vi "get mcs registers.vi"(11 "MCS CSV":string[][](array[string])) -> (0 "coils":T1(array[cluster]), 1 "Array 2":i32[][](array[numeric]), 2 "Array 3":i32[][](array[numeric]), 3 "Array 4":i32[][](array[numeric]), 4 "Array":T2[][](array[typedef]))   [LabVIEW 2025]
uses:
  mcs/Tachometer_MAIN Folder/CTRLS/New/MCS Tag.ctl
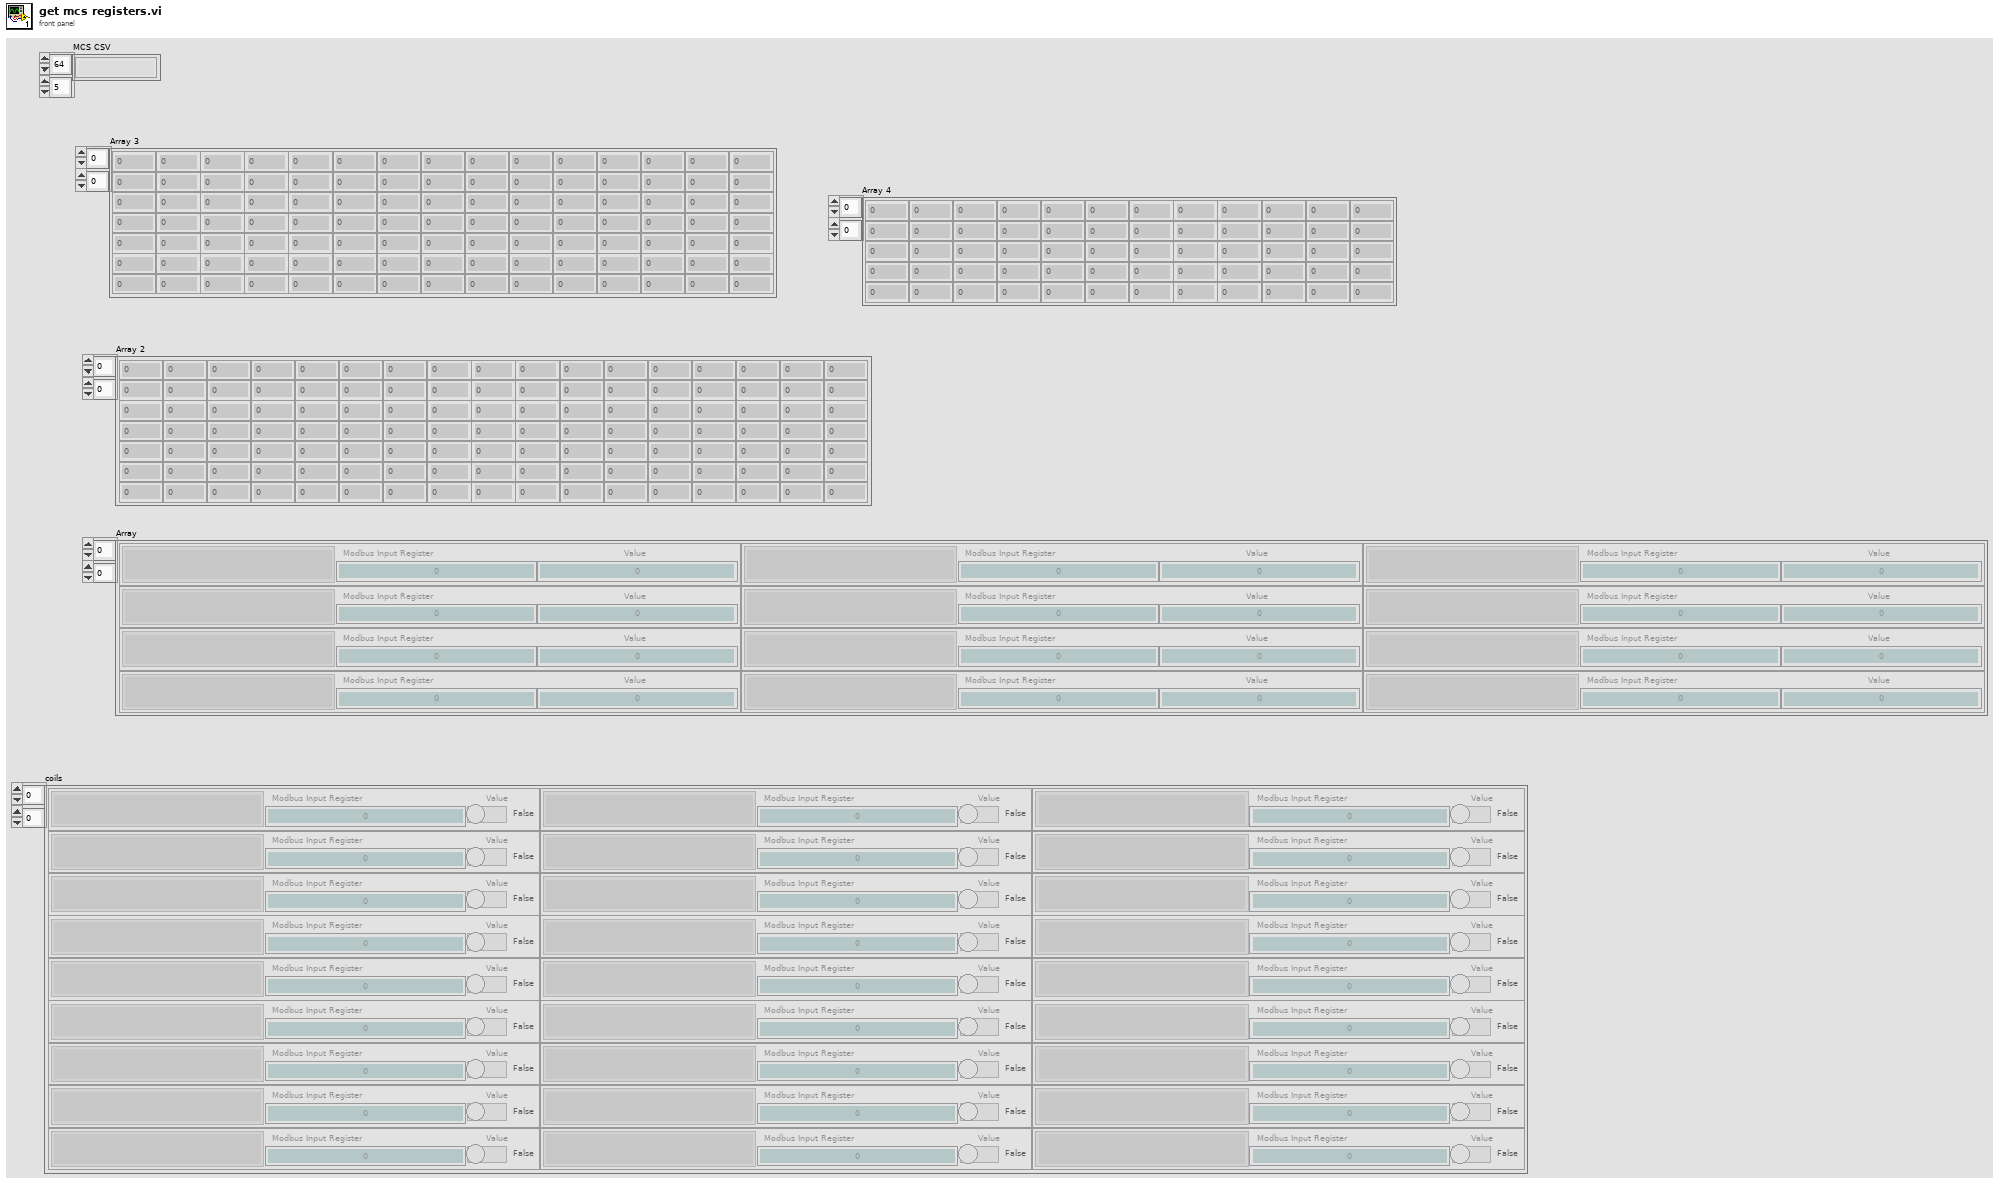
[diagram p1: front panel]
types:
  T1 = cluster{"Tag Name":string, "Modbus Input Register":sgl, "Value":bool}[][]
  T2 = typedef "MCS Tag.ctl" = cluster{"Tag Name":string, "Modbus Input Register":sgl, "Value":sgl}
  T3 = cluster{"Tag Name":string, "Modbus Input Register":sgl, bool}
  T4 = cluster{"Tag Name":string, "Modbus Input Register":sgl, bool}[]
  T5 = cluster{"Tag Name":string, "Modbus Input Register":sgl, bool}[][]
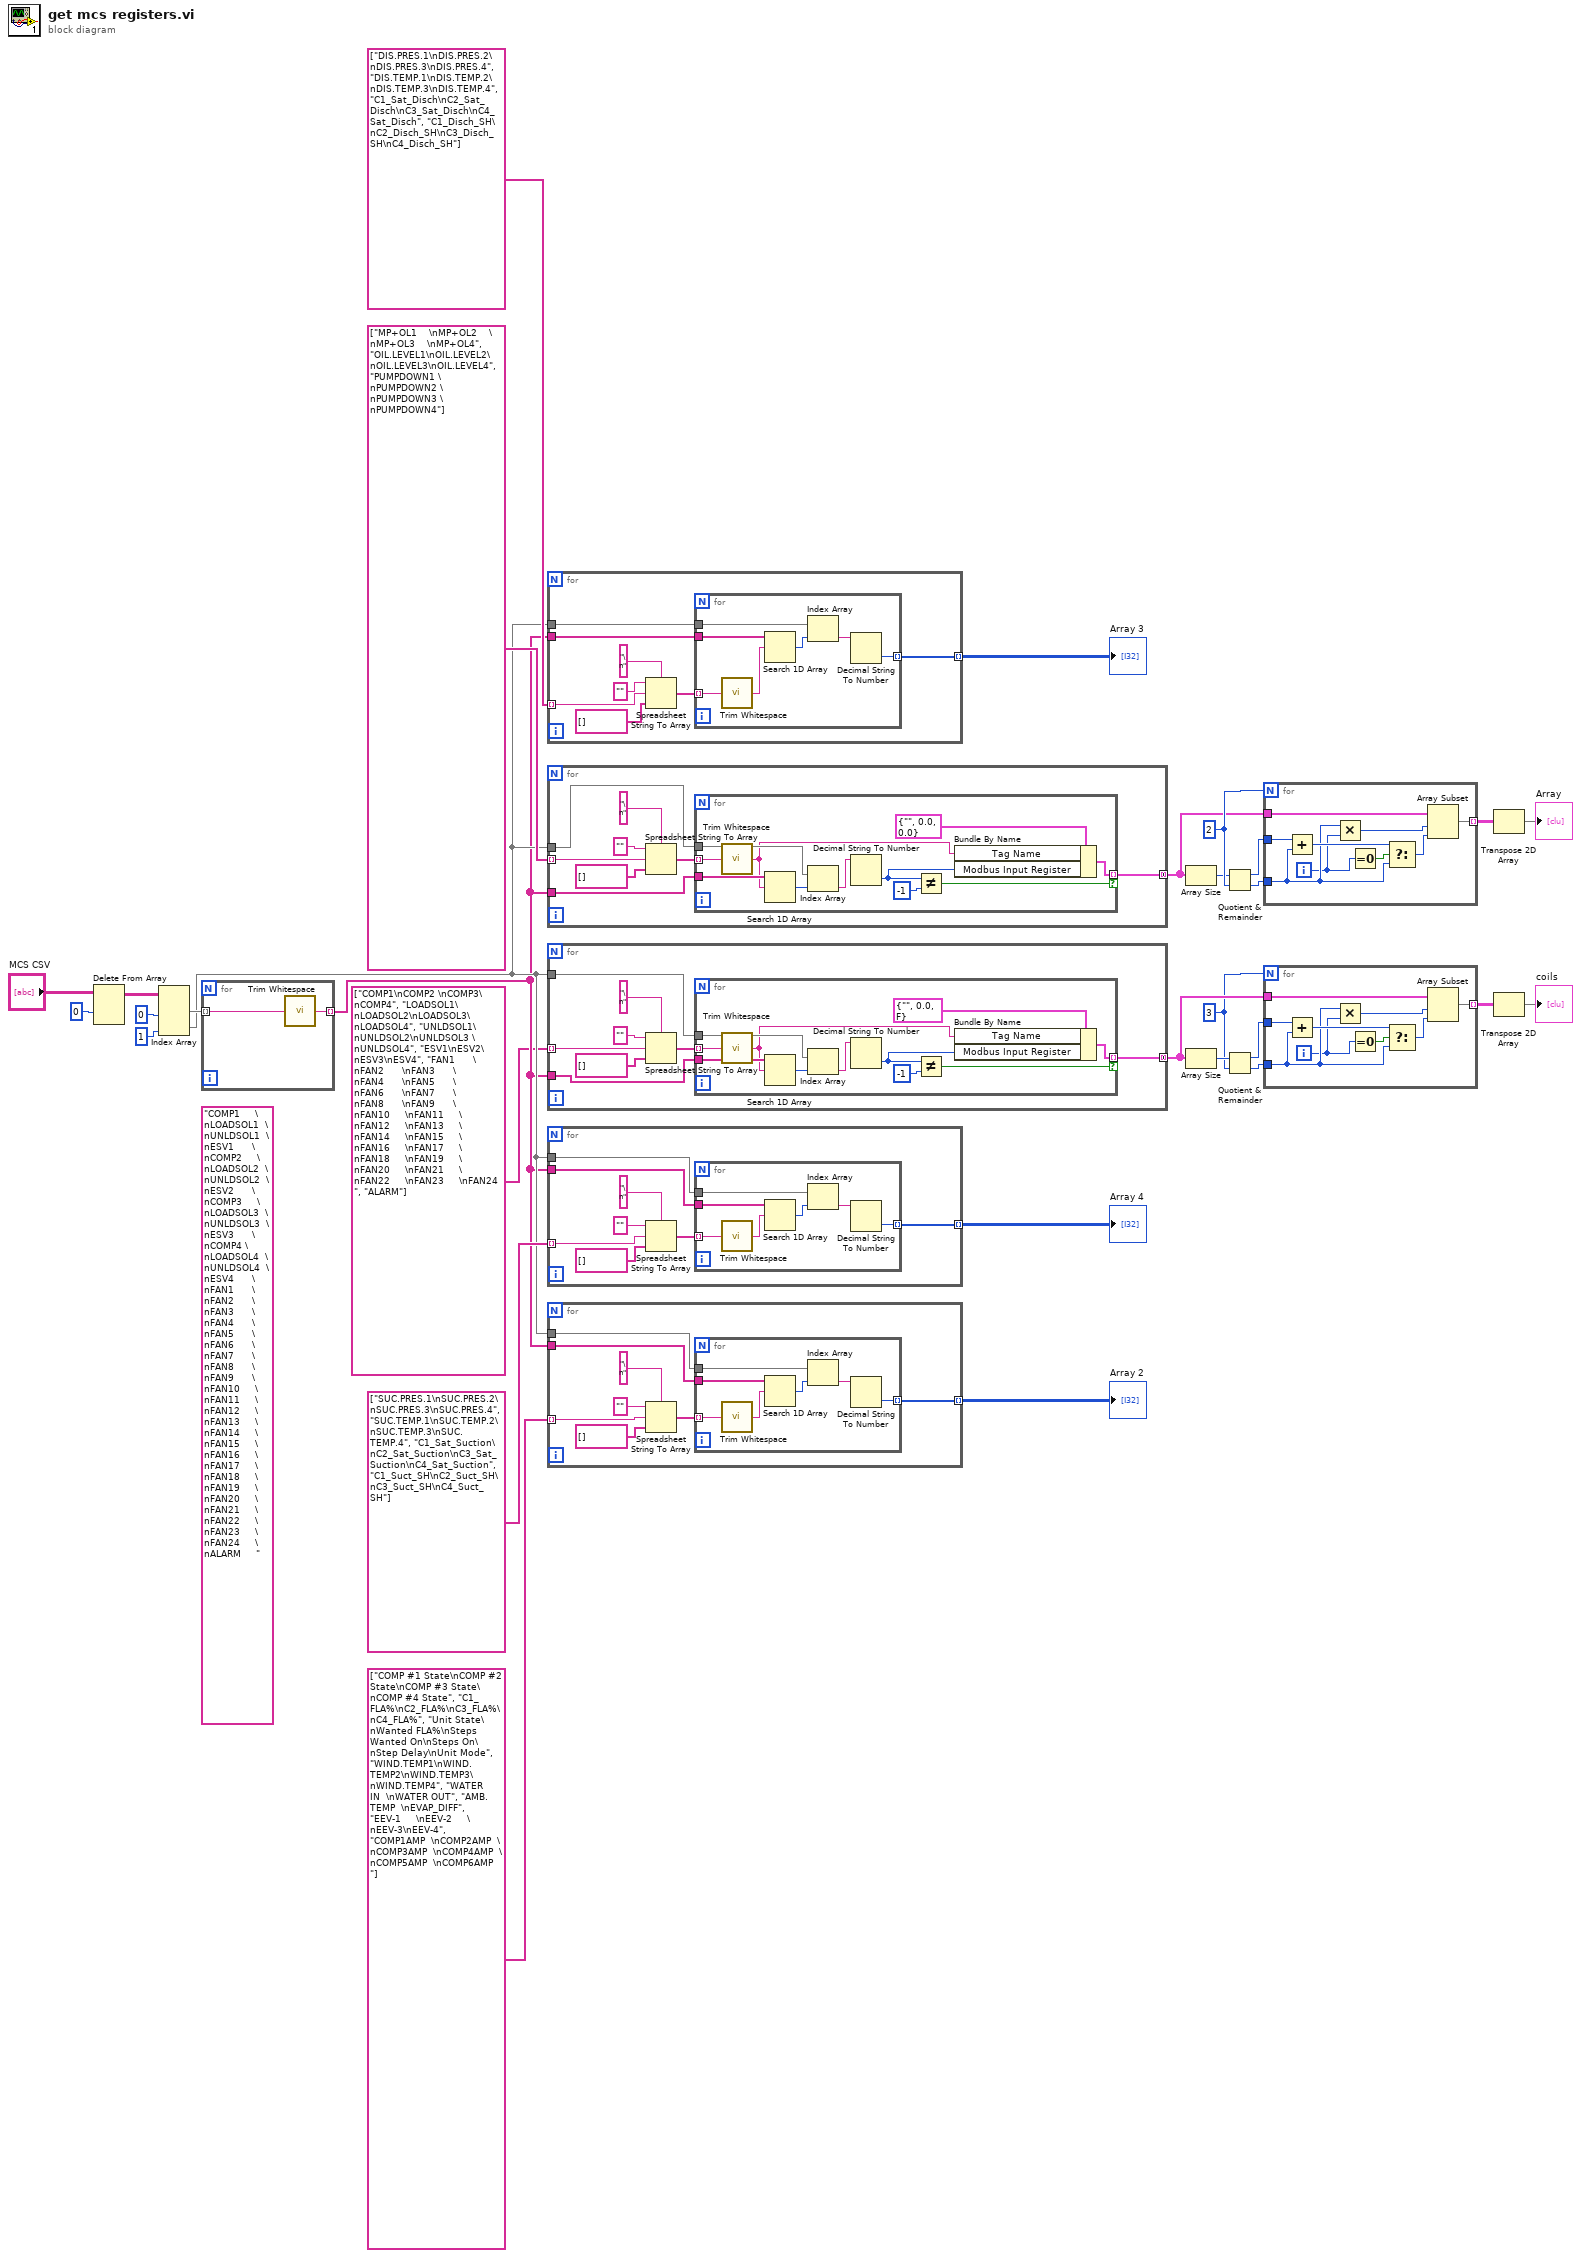
[diagram p0: block diagram]
diagram:
  w5 = 2
  w10 = 3
  (unwired) "COMP1     \nLOADSOL1  \nUNLDSOL1  \nESV1      \nCOMP2     \nLOADSOL2  \nUNLDSOL2  \nESV2      \nCOMP3     \nLOADSOL3  \nUNLDSOL3  \nESV3      \nCOMP4 \nLOADSOL4  \nUNLDSOL4  \nESV4      \nFAN1      \nFAN2      \nFAN3      \nFAN4      \nFAN5      \nFAN6      \nFAN7      \nFAN8      \nFAN9      \nFAN10     \nFAN11     \nFAN12     \nFAN13     \nFAN14     \nFAN15     \nFAN16     \nFAN17     \nFAN18     \nFAN19     \nFAN20     \nFAN21     \nFAN22     \nFAN23     \nFAN24     \nALARM     "
  n1 = Delete From Array(array="MCS CSV", index (row)=0) -> (array with subset deleted=w20:string[][])  [unwired: 2 in, 1 out]
  n2 = Index Array(array=w20, index (col) #1=0 ("disabled index (col)"), index (col) #2=1 ("index (col)")) -> (element #1=w21:string[], element #2=w14:string[])  [unwired: 2 in]
  n3 = for {
    tunnel: [w32] -> w13 mode=indexing
    tunnel: w21 -> [w31] mode=indexing
    n4 = call-poly <vilib>:"Trim Whitespace.vi"("string"=w31) -> ("trimmed string"=w32:string)  [unwired: 1 in]
  }
  n5 = for {
    tunnel: w13 -> [w36]
    tunnel: w14 -> [w35]
    tunnel: string[] ["DIS.PRES.1\nDIS.PRES.2\nDIS.PRES.3\nDIS.PRES.4", "DIS.TEMP.1\nDIS.TEMP.2\nDIS.TEMP.3\nDIS.TEMP.4", "C1_Sat_Disch\nC2_Sat_Disch\nC3_Sat_Disch\nC4_Sat_Disch", "C1_Disch_SH\nC2_Disch_SH\nC3_Disch_SH\nC4_Disch_SH"] -> [w33] mode=indexing
    tunnel: [w34] -> w27 mode=indexing
    n6 = Spreadsheet String To Array(delimiter (Tab)="\n", format string="", spreadsheet string=w33, array type (2D Dbl)=string[] []) -> (array=w37:string[])
    n7 = for {
      tunnel: w37 -> [w47] mode=indexing
      tunnel: w35 -> [w43]
      tunnel: w36 -> [w42]
      tunnel: [w41] -> w34 mode=indexing
      n8 = call-poly <vilib>:"Trim Whitespace.vi"("string"=w47) -> ("trimmed string"=w46:string)  [unwired: 1 in]
      n9 = Search 1D Array(1D array=w42, element=w46) -> (index of element=w45:i32)  [unwired: 1 in]
      n10 = Index Array(array=w43, index=w45) -> (element=w44:string)
      n11 = Decimal String To Number(string=w44) -> (number=w41:i32)  [unwired: 2 in, 1 out]
    }
  }
  "Array 3" <- w27
  n12 = for {
    tunnel: w13 -> [w51]
    tunnel: w14 -> [w50]
    tunnel: string[] ["MP+OL1    \nMP+OL2    \nMP+OL3    \nMP+OL4", "OIL.LEVEL1\nOIL.LEVEL2\nOIL.LEVEL3\nOIL.LEVEL4", "PUMPDOWN1 \nPUMPDOWN2 \nPUMPDOWN3 \nPUMPDOWN4"] -> [w49] mode=indexing
    tunnel: [w48] -> w1 mode=concatenating
    n13 = Spreadsheet String To Array(delimiter (Tab)="\n", format string="", spreadsheet string=w49, array type (2D Dbl)=string[] []) -> (array=w52:string[])
    n14 = for {
      tunnel: w52 -> [w66] mode=indexing
      tunnel: w50 -> [w63]
      tunnel: w51 -> [w62]
      tunnel: [w60] -> w48 mode=indexing if=w56
      n15 = call-poly <vilib>:"Trim Whitespace.vi"("string"=w66) -> ("trimmed string"=w61:string)  [unwired: 1 in]
      n16 = Search 1D Array(1D array=w62, element=w61) -> (index of element=w65:i32)  [unwired: 1 in]
      n17 = Index Array(array=w63, index=w65) -> (element=w64:string)
      n18 = Decimal String To Number(string=w64) -> (number=w58:i32)  [unwired: 2 in, 1 out]
      n19 = Not Equal?(x=w58, y=-1) -> (x != y?=w56:bool)
      n20 = Bundle By Name(cluster=T2 {"Tag Name"="", "Modbus Input Register"=0.0, "Value"=0.0} ("MCS Tag"), "Tag Name"=w61, "Modbus Input Register"=w58) -> (w60:T2)
    }
  }
  n21 = for {
    tunnel: w13 -> [w70]
    tunnel: w14 -> [w69]
    tunnel: string[] ["COMP1\nCOMP2 \nCOMP3\nCOMP4", "LOADSOL1\nLOADSOL2\nLOADSOL3\nLOADSOL4", "UNLDSOL1\nUNLDSOL2\nUNLDSOL3 \nUNLDSOL4", "ESV1\nESV2\nESV3\nESV4", "FAN1      \nFAN2      \nFAN3      \nFAN4      \nFAN5      \nFAN6      \nFAN7      \nFAN8      \nFAN9      \nFAN10     \nFAN11     \nFAN12     \nFAN13     \nFAN14     \nFAN15     \nFAN16     \nFAN17     \nFAN18     \nFAN19     \nFAN20     \nFAN21     \nFAN22     \nFAN23     \nFAN24  ", "ALARM"] -> [w68] mode=indexing
    tunnel: [w67] -> w15 mode=concatenating
    n22 = Spreadsheet String To Array(delimiter (Tab)="\n", format string="", spreadsheet string=w68, array type (2D Dbl)=string[] []) -> (array=w71:string[])
    n23 = for {
      tunnel: w71 -> [w85] mode=indexing
      tunnel: w69 -> [w82]
      tunnel: w70 -> [w81]
      tunnel: [w79] -> w67 mode=indexing if=w75
      n24 = call-poly <vilib>:"Trim Whitespace.vi"("string"=w85) -> ("trimmed string"=w80:string)  [unwired: 1 in]
      n25 = Search 1D Array(1D array=w81, element=w80) -> (index of element=w84:i32)  [unwired: 1 in]
      n26 = Index Array(array=w82, index=w84) -> (element=w83:string)
      n27 = Decimal String To Number(string=w83) -> (number=w77:i32)  [unwired: 2 in, 1 out]
      n28 = Not Equal?(x=w77, y=-1) -> (x != y?=w75:bool)
      n29 = Bundle By Name(cluster=T3 {"Tag Name"="", "Modbus Input Register"=0.0, FALSE} ("MCS Tag"), "Tag Name"=w80, "Modbus Input Register"=w77) -> (w79:T3)
    }
  }
  n30 = for {
    tunnel: w13 -> [w89]
    tunnel: w14 -> [w88]
    tunnel: string[] ["SUC.PRES.1\nSUC.PRES.2\nSUC.PRES.3\nSUC.PRES.4", "SUC.TEMP.1\nSUC.TEMP.2\nSUC.TEMP.3\nSUC.TEMP.4", "C1_Sat_Suction\nC2_Sat_Suction\nC3_Sat_Suction\nC4_Sat_Suction", "C1_Suct_SH\nC2_Suct_SH\nC3_Suct_SH\nC4_Suct_SH"] -> [w86] mode=indexing
    tunnel: [w87] -> w25 mode=indexing
    n31 = Spreadsheet String To Array(delimiter (Tab)="\n", format string="", spreadsheet string=w86, array type (2D Dbl)=string[] []) -> (array=w90:string[])
    n32 = for {
      tunnel: w90 -> [w100] mode=indexing
      tunnel: w88 -> [w96]
      tunnel: w89 -> [w95]
      tunnel: [w94] -> w87 mode=indexing
      n33 = call-poly <vilib>:"Trim Whitespace.vi"("string"=w100) -> ("trimmed string"=w99:string)  [unwired: 1 in]
      n34 = Search 1D Array(1D array=w95, element=w99) -> (index of element=w98:i32)  [unwired: 1 in]
      n35 = Index Array(array=w96, index=w98) -> (element=w97:string)
      n36 = Decimal String To Number(string=w97) -> (number=w94:i32)  [unwired: 2 in, 1 out]
    }
  }
  "Array 4" <- w25
  n37 = for {
    tunnel: w13 -> [w104]
    tunnel: w14 -> [w103]
    tunnel: string[] ["COMP #1 State\nCOMP #2 State\nCOMP #3 State\nCOMP #4 State", "C1_FLA%\nC2_FLA%\nC3_FLA%\nC4_FLA%", "Unit State\nWanted FLA%\nSteps Wanted On\nSteps On\nStep Delay\nUnit Mode", "WIND.TEMP1\nWIND.TEMP2\nWIND.TEMP3\nWIND.TEMP4", "WATER IN  \nWATER OUT", "AMB.TEMP  \nEVAP_DIFF", "EEV-1     \nEEV-2     \nEEV-3\nEEV-4", "COMP1AMP  \nCOMP2AMP  \nCOMP3AMP  \nCOMP4AMP  \nCOMP5AMP  \nCOMP6AMP  "] -> [w101] mode=indexing
    tunnel: [w102] -> w29 mode=indexing
    n38 = Spreadsheet String To Array(delimiter (Tab)="\n", format string="", spreadsheet string=w101, array type (2D Dbl)=string[] []) -> (array=w105:string[])
    n39 = for {
      tunnel: w105 -> [w115] mode=indexing
      tunnel: w103 -> [w111]
      tunnel: w104 -> [w110]
      tunnel: [w109] -> w102 mode=indexing
      n40 = call-poly <vilib>:"Trim Whitespace.vi"("string"=w115) -> ("trimmed string"=w114:string)  [unwired: 1 in]
      n41 = Search 1D Array(1D array=w110, element=w114) -> (index of element=w113:i32)  [unwired: 1 in]
      n42 = Index Array(array=w111, index=w113) -> (element=w112:string)
      n43 = Decimal String To Number(string=w112) -> (number=w109:i32)  [unwired: 2 in, 1 out]
    }
  }
  "Array 2" <- w29
  n44 = Array Size(array=w1) -> (size(s)=w4:i32)
  n45 = Array Size(array=w15) -> (size(s)=w11:i32)
  n46 = Quotient & Remainder(x=w4, y=w5) -> (x-y*floor(x/y)=w7:i32, floor(x/y)=w6:i32)
  n47 = Quotient & Remainder(x=w11, y=w10) -> (x-y*floor(x/y)=w8:i32, floor(x/y)=w9:i32)
  n48 = for {
    N: w5 -> [_]
    tunnel: w1 -> [w124]
    tunnel: [w123] -> w3 mode=indexing
    tunnel: w6 -> [w118]
    tunnel: w7 -> [w120]
    i -> [w116]
    n49 = Add(x=w120, y=w118) -> (x+y=w119:i32)
    n50 = Multiply(x=w118, y=w116) -> (x*y=w122:i32)
    n51 = Equal To 0?(x=w116) -> (x = 0?=w121:bool)
    n52 = Select(t=w119, s=w121, f=w118) -> (s? t:f=w117:i32)
    n53 = Array Subset(array=w124, index=w122, length=w117) -> (w123:T2[])
  }
  n54 = for {
    N: w10 -> [_]
    tunnel: w15 -> [w133]
    tunnel: [w132] -> w16 mode=indexing
    tunnel: w9 -> [w127]
    tunnel: w8 -> [w129]
    i -> [w125]
    n55 = Add(x=w129, y=w127) -> (x+y=w128:i32)
    n56 = Multiply(x=w127, y=w125) -> (x*y=w131:i32)
    n57 = Equal To 0?(x=w125) -> (x = 0?=w130:bool)
    n58 = Select(t=w128, s=w130, f=w127) -> (s? t:f=w126:i32)
    n59 = Array Subset(array=w133, index=w131, length=w126) -> (w132:T4)
  }
  n60 = Transpose 2D Array(2D array=w3) -> (transposed array=→"Array":T2[][])
  n61 = Transpose 2D Array(2D array=w16) -> (transposed array=→"coils":T5)
